vi "FuncVI_Sub - Script - Read and Write Parameter.vi"(5 "cmd (read)":enum16{"create", "destroy", "write", "read"}(ring)=enum."read", 6 "var type":u32=128, 7 "VC Handle":T1=-1, 8 "error in":errorcluster, 9 "writer ID":u32, 10 "flattened value":string, 11 "var name/const":string) -> (0 "error out":errorcluster, 1 "constant?":bool, 2 "flattened value out":string, 3 "dup var name/const":string, 4 "var type out":u32)   [LabVIEW 2021]
doc: "::: CalcExpress Toolkit :::\nCopyright (c) 2000-2026 Konstantin Shifershteyn. All rights reserved."
uses:
  cetypes.llb/VarMan Variable Context Handle.ctl
  cetypes.llb/CalcExpress Data Type.ctl
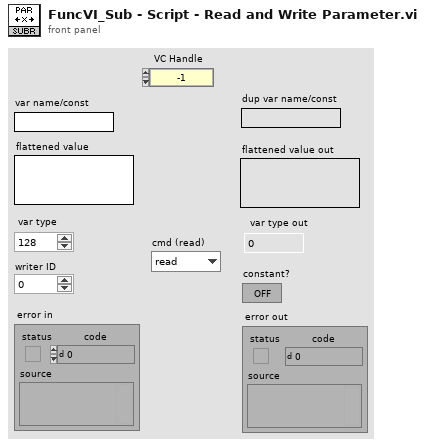
[diagram p1: front panel]
types:
  T1 = typedef "VarMan Variable Context Handle.ctl" = i32
  T2 = typedef "CalcExpress Data Type.ctl" = enum32{"String", "DBL Number", "identifier", "1D Array of DBL", "2D Array of DBL", "CDB Number", "1D Array of CDB", "2D Array of CDB", "1D Array of String", "2D Array of String", "Unknown data type"}
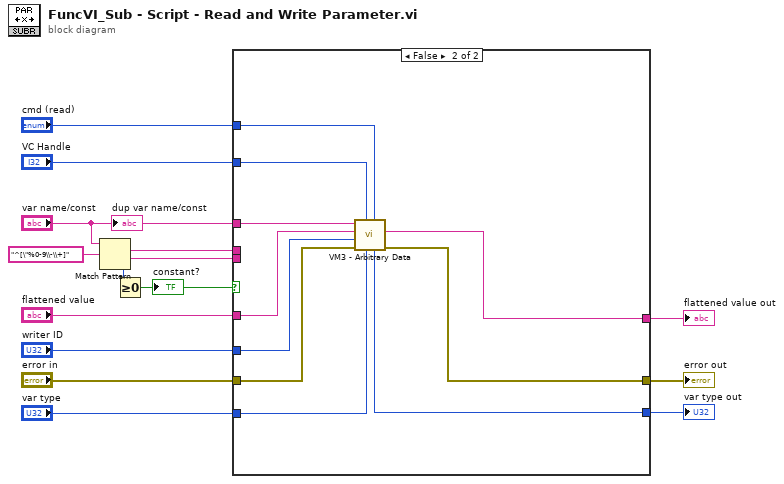
[diagram p0: block diagram]
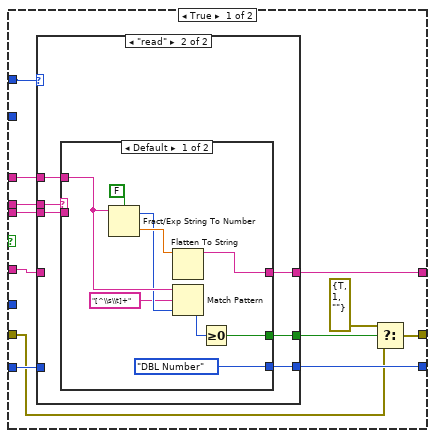
[diagram p2: hidden frame]
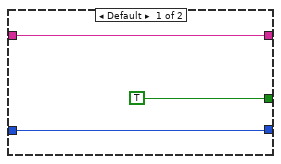
[diagram p3: hidden frame]
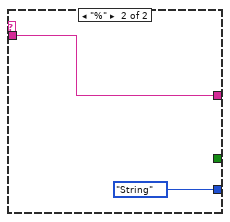
[diagram p4: hidden frame]
diagram:
  n1 = Match Pattern(string="var name/const", regular expression="^[\"%0-9\\-\\+]") -> (match substring=w7:string, after substring=w3:string, offset past match=w6:i32)  [unwired: 1 in, 1 out]
  n2 = Greater Or Equal To 0?(x=w6) -> (x >= 0?=w5:bool)
  "constant?" <- w5
  n3 = case shown="False" w5 {
    tunnel: "var name/const" -> [w26 w57]
    tunnel: "flattened value" -> [w22 w56]
    tunnel: "error in" -> [w17 w55]
    tunnel: "var type" -> [w23 w54]
    tunnel: [w24 w53] -> w11
    tunnel: [w18 w52] -> w10
    tunnel: [w25 w51] -> w9
    tunnel: "VC Handle" -> [_ w50]
    tunnel: w7 -> [w27 _]
    tunnel: w3 -> [w21 _]
    tunnel: "cmd (read)" -> [w16 w49]
    tunnel: "writer ID" -> [_ w48]
    frame True {
      n4 = case shown="\"read\"" w16 {
        tunnel: w27 -> [_ w36]
        tunnel: w26 -> [_ w32]
        tunnel: [w29 w35] -> w25
        tunnel: [w30 w34] -> w24
        tunnel: w23 -> [w30 _]
        tunnel: w22 -> [w29 _]
        tunnel: w21 -> [_ w33]
        tunnel: [TRUE w31] -> w19
        frame Default {
        }
        frame "read" {
          n5 = case shown="Default" w36 {
            tunnel: w32 -> [w41 _]
            tunnel: [w44 w46] -> w35
            tunnel: [CalcExpress_Data_Type."DBL Number" ("data type") CalcExpress_Data_Type."String" ("data type")] -> w34
            tunnel: w33 -> [_ w46]
            tunnel: [w38 _] -> w31
            frame Default {
              n6 = Fract/Exp String To Number(use system decimal point (T)=FALSE, string=w41) -> (offset past number=w40:i32, number=w42:dbl)  [unwired: 2 in]
              n7 = Flatten To String(anything=w42) -> (data string=w44:string)  [unwired: 3 in, 2 out]
              n8 = Match Pattern(string=w41, regular expression="[^\\s\\t]+", offset (0)=w40) -> (offset past match=w37:i32)  [unwired: 3 out]
              n9 = Greater Or Equal To 0?(x=w37) -> (x >= 0?=w38:bool)
            }
            frame "%" {
            }
          }
        }
      }
      n10 = Select(t=errorcluster {"status"=TRUE, "code"=1, "source"=""}, s=w19, f=w17) -> (s? t:f=w18:errorcluster)
    }
    frame False {
      n11 = call "VM3 - Arbitrary Data.vi"("cmd (read)"=w49, "var type in"=w54, "VC Handle"=w50, "error in"=w55, "writer ID"=w48, "flattened value in"=w56, "name_spec"=w57) -> ("error out"=w52:errorcluster, "flattened value out"=w51:string, "var type out"=w53:u32)  [unwired: 2 out]
    }
  }
  "var type out" <- w11
  "error out" <- w10
  "flattened value out" <- w9
  "dup var name/const" <- "var name/const"
